vi "CE Math - Timer.vi"(6 "error in (no error)":errorcluster, 9 "ticks in":u32) -> (0 "error out":errorcluster, 3 "ticks out":u32)   [LabVIEW 2021]
doc: "::: CalcExpress Toolkit :::\nCopyright (c) 2000-2026 Konstantin Shifershteyn. All rights reserved."
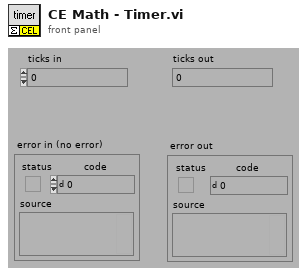
[diagram p1: front panel]
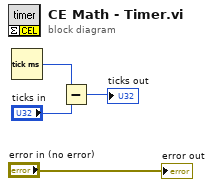
[diagram p0: block diagram]
diagram:
  n1 = Tick Count (ms)() -> (millisecond timer value=w2:u32)
  n2 = Subtract(x=w2, y="ticks in") -> (x-y=→"ticks out":u32)
  "error out" <- "error in (no error)"
